vi "4Pi Focus Lock.vi"() -> ()   [LabVIEW 2016]
uses:
  4Pi Focus Lock Controls/4Pi Focus Lock - Notifier Type.ctl
  4Pi Focus Lock Controls/4Pi Focus Lock - Actions.ctl
  <vilib>/vision/Image Controls.llb/IMAQ Image.ctl
  Hardware Configuration/Hardware Configuration Controls/Device Type.ctl
  Hardware Configuration/Hardware Configuration Controls/Device Function.ctl
  Device Library/Cameras/Camera Controls/Generic Camera ROI.ctl
  Device Library/Cameras/Camera Controls/Generic Camera Actions.ctl
  Device Library/Stages/Stages Controls/Stage Actions.ctl
  <vilib>/addons/control/pid/pid.llb/PID (DBL).vi
  <vilib>/addons/control/pid/NI_PID_pid.lvlib
  <vilib>/vision/NI_Vision_Development_Module.lvlib
panel:
  out "CC Max":cluster{" cc max":dbl}(graph)
  in  "Pixe Size (µm)":dbl=2.0
  out "X Y Fit Value (µm)":cluster{dbl, dbl, dbl}(graph)
  out "cc max":dbl=1.0 format="%.3g"
  out "Target X Position cc (px)":dbl=1.0 format="%.3g"
  out "Target Y Position cc (px)":dbl=1.0 format="%.3g"
  out "Measured Y Position cc (px)":dbl=1.0 format="%.3g"
  out "Measured X Position cc (px)":dbl=1.0 format="%.3g"
  in  "Z Correction Active":bool=TRUE
  in  "Frame Accumulation":u32=1
  in  "Z Drift Threshold (µm)":dbl=2.0
  in  "Z Move Limit (µm)":dbl=2.0
  out "Z Move":bool
  in  "Update Scale Factor":dbl=2.0
  out "dz (µm)":dbl format="%.2f"
  out "dt (s)":dbl format="%.3f"
  out "Measured Z (µm)":dbl=1.0 format="%.3g"
  out "Target Z (µm)":dbl=1.0 format="%.3g"
  out "Stage Position (µm)":dbl=1.0 format="%.2g"
  in  "Quit":bool
  in  "Sample Z Step No.":u32=2
  in  "Sample Z Step Size (µm)":dbl=2.0
  in  "D (Derivative)":dbl
  in  "I (Integral)":dbl
  in  "P (Proportional)":dbl=2.0
  in  "Set Camera ROI":bool
  out "Z Target and Fit Value (µm)":T1(graph)
  in  "Start Lock":bool
  # "PID Control Values"
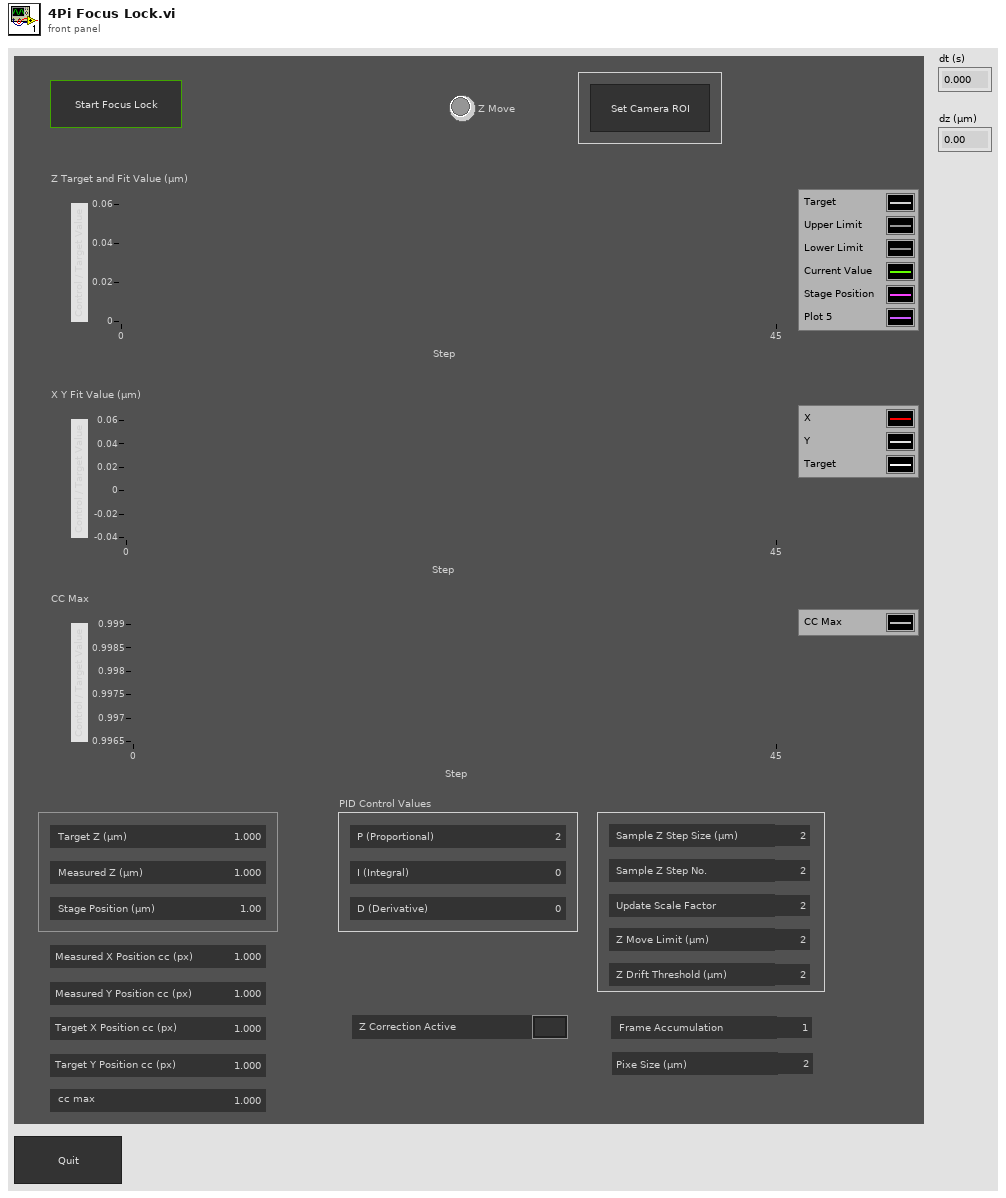
[diagram p1: front panel]
types:
  T1 = cluster{"Target 01":dbl, dbl, dbl, "Current 01":dbl, "Stage Position":dbl}
  T2 = typedef "4Pi Focus Lock - Actions.ctl" = enum16{"Idle", "Start Lock", "Restart Lock", "Get Target Position", "Get Ref Stack", "Cal Ref FFT", "Move To Init Z", "Start Primary Camera", "Get Current Position", "Get Current XY Position", "Get Current Position 1", "Get Actual Position", "Check Drift", "Move Z", "Update Plots", "Delay", "Abort", "Exit Loop", "Quit"}
  T3 = typedef "4Pi Focus Lock - Notifier Type.ctl" = cluster{"Actions":T2, "Z Drift Threshold":dbl, "Z Stage Move Limit (µm)":dbl, "Abort If Error":bool, "Z Correction Active":bool, "PID Values":dbl[], "Running?":bool, "Update Delay (ms)":i32, "Z Step Size (µm)":dbl, "Z Step No.":u32, "No. of Frames":u32, "Ref Stack (SGL)":T4[], "Cur Image (SGL)":T4, "CC Image (SGL) ":T4, "Sample Z (µm)":dbl[], "Initial Z Position (µm)":dbl, "Ref FFT Stack (CSG)":T4[], "Tmp Image FFT (CSG) ":T4[], "CC Image Max (SGL)":T4}
  T4 = typedef "IMAQ Image.ctl" = refnum<image>
  T5 = typedef "Image Type" = u32
  T6 = typedef "Device Function.ctl" = enum16{"Primary", "Secondary", "Overview", "Wide Field Drift Correction", "642 nm Excitation", "560 nm Excitation", "940 nm Excitation", "546 nm Excitation", "488 nm Excitation", "405 nm Excitation", "Objective Drift Correction", "4Pi Focus Lock", "4Pi Objective Lock", "Objective XY", "Objective Z", "Sample XY", "Sample Coarse Z", "Sample Z", "4Pi Lower", "4Pi Upper", "Em Small", "Em Large", "Ex Small", "Ex Large", "Mojo", "Adj Cavity", "Line Scanning", "Alert"}
  T7 = typedef "Device Type.ctl" = enum16{"AOTF", "Camera", "Deformable Mirror", "Laser", "Flip Mirror", "Shutter", "Stage", "Waveform", "FPGA", "Email"}
  T8 = typedef "Stage Actions.ctl" = enum16{"Get Position", "MVR", "MOVE", "HALT", "ONTARGET", "ERROR", "REFERENCE", "INIT", "VELOCITY", "STATUS", "EXIT", "HOME", "ZEROPOS", "NANOPOS", "ANALOG", "QUIT"}
  T9 = typedef "Generic Camera Actions.ctl" = enum16{"Status", "Live Preview", "Capture", "Abort", "Set Exposure Time (s)", "Get Exposure Time (s)", "Record Settings", "Set ROI", "Get ROI", "Defect Correction On/Off", "Cooler On/Off", "Fan On/Off", "Quit"}
  T10 = typedef "Generic Camera ROI.ctl" = cluster{"H_Offset":u16, "V_Offset":u16, "H_Width":u16, "V_Width":u16}
  T11 = typedef "Stage Status.ctl" = enum16{"Error", "Abort", "Busy", "On Target"}
  T12 = typedef "2D Gaussian - Best Fit Parameters.ctl" = cluster{"Amplitude":dbl, "X Position":dbl, "Y Position":dbl, "X Width":dbl, "Y Width":dbl, "Offset":dbl}
  T13 = cluster{"PID Values[0]":dbl, "PID Values[1]":dbl, "PID Values[2]":dbl}
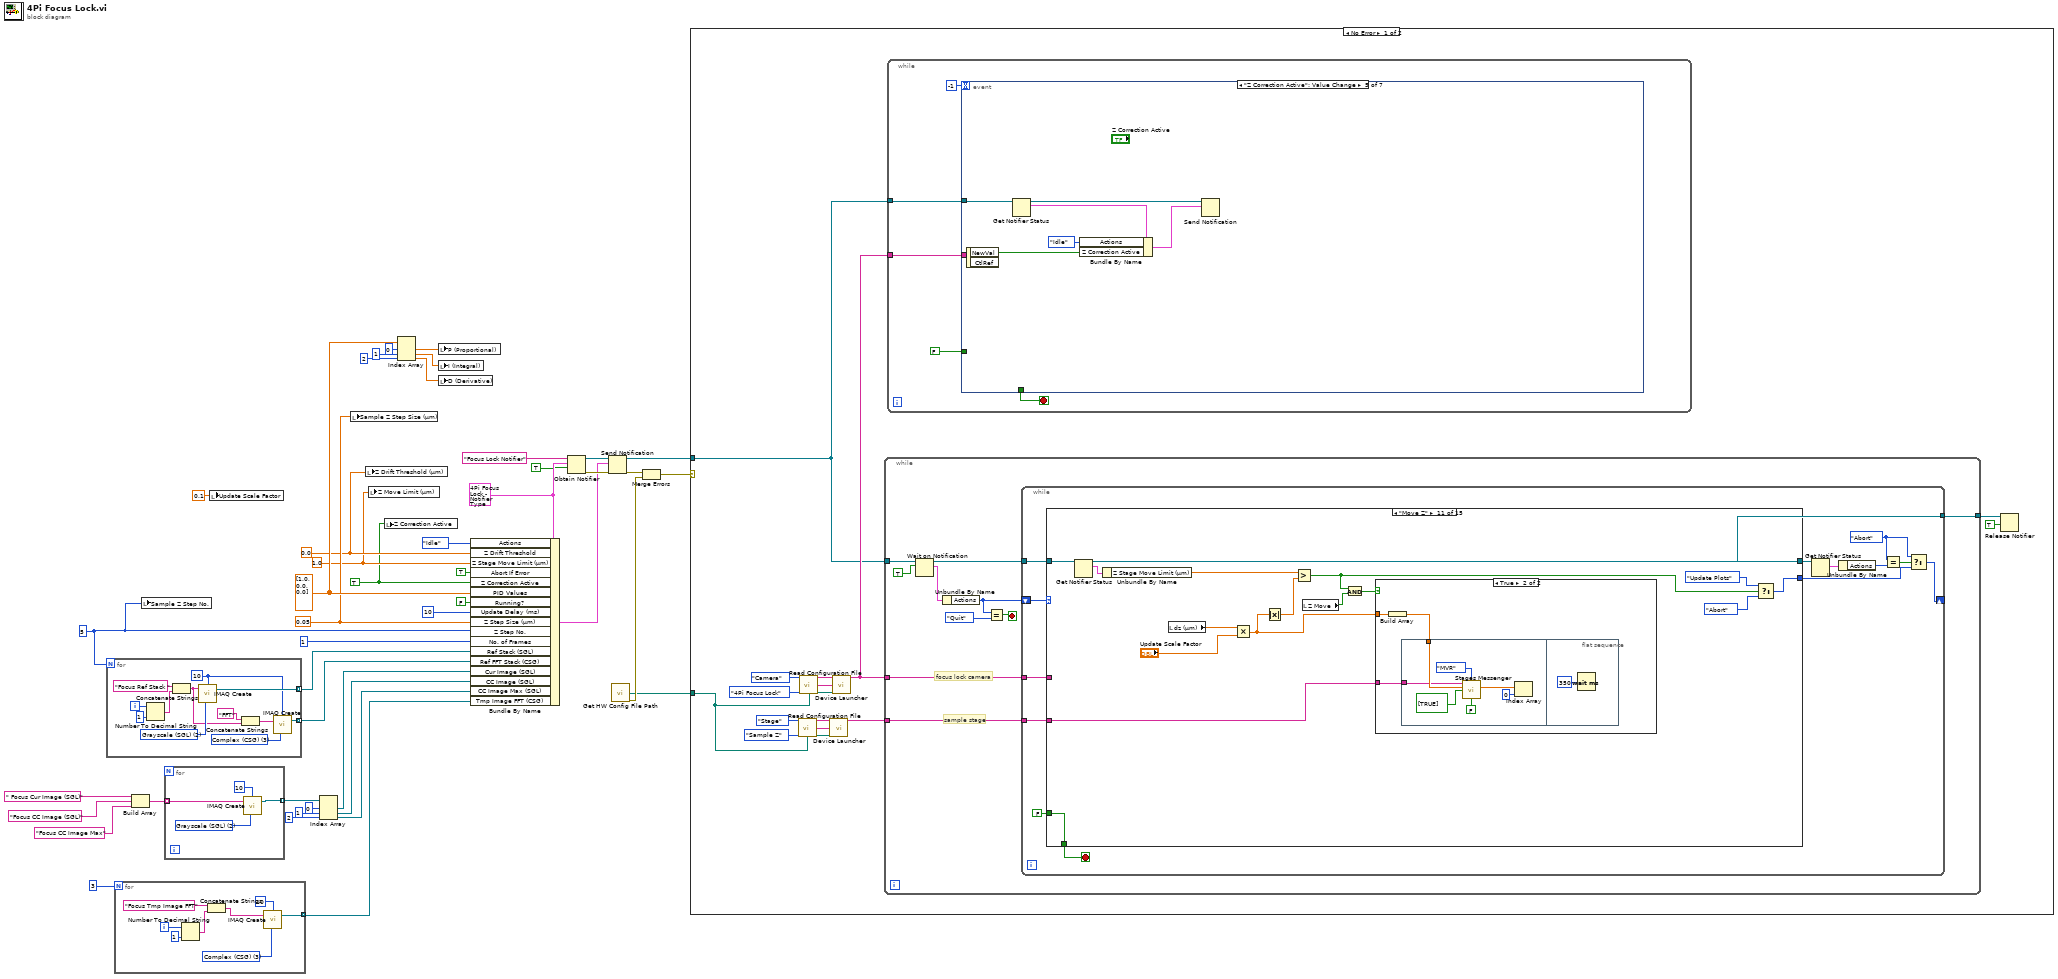
[diagram p0: block diagram]
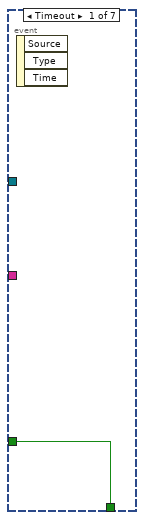
[diagram p2: hidden frame]
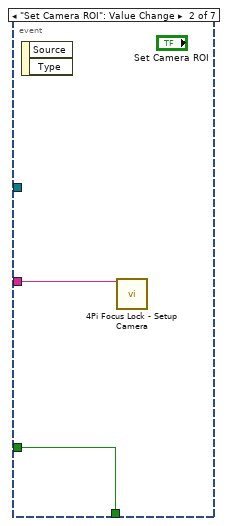
[diagram p3: hidden frame]
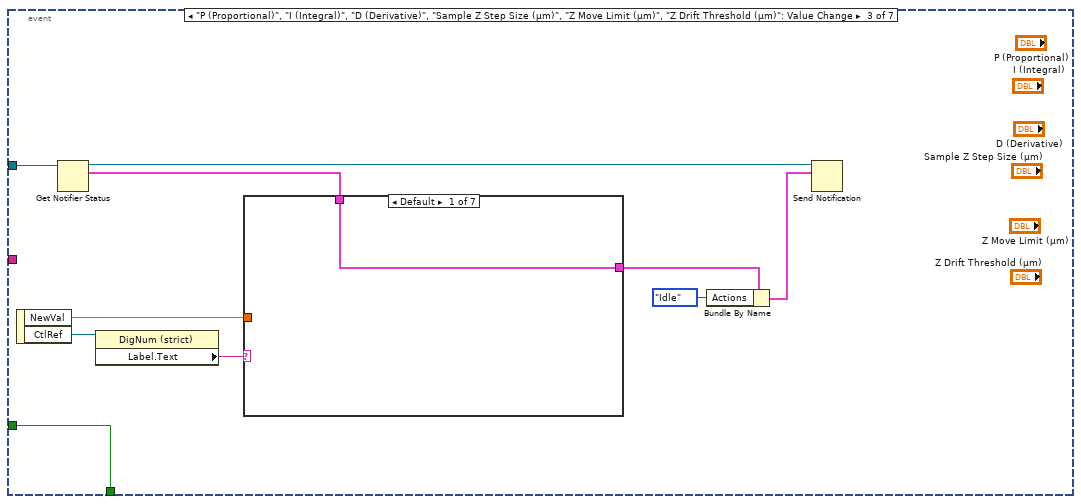
[diagram p4: hidden frame]
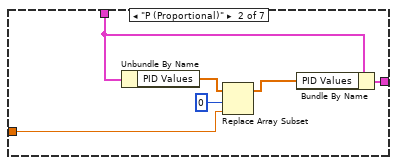
[diagram p5: hidden frame]
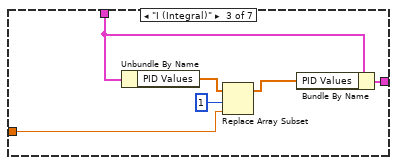
[diagram p6: hidden frame]
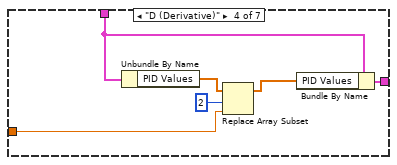
[diagram p7: hidden frame]
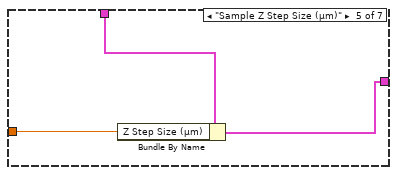
[diagram p8: hidden frame]
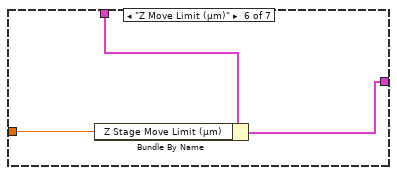
[diagram p9: hidden frame]
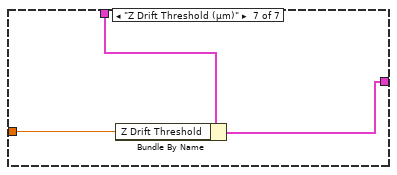
[diagram p10: hidden frame]
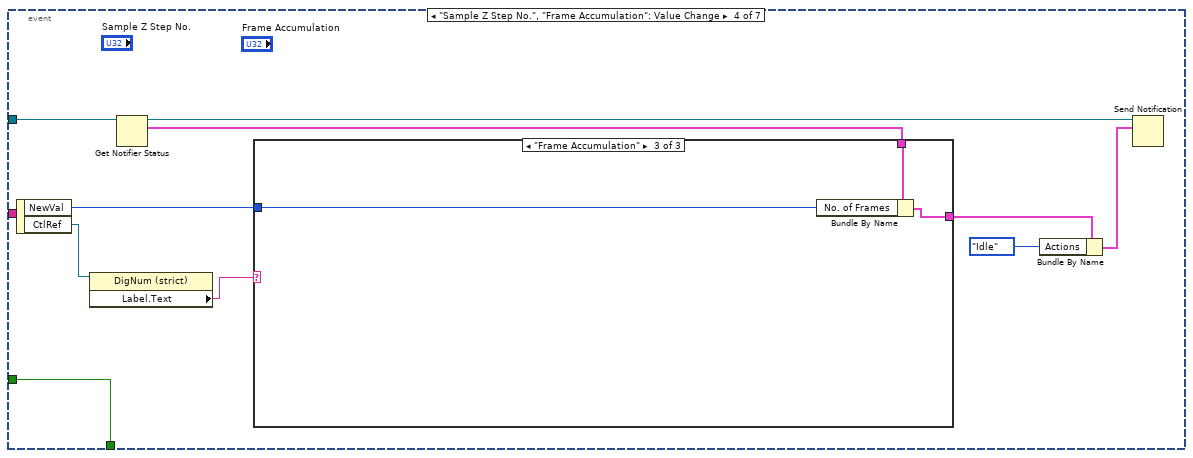
[diagram p11: hidden frame]
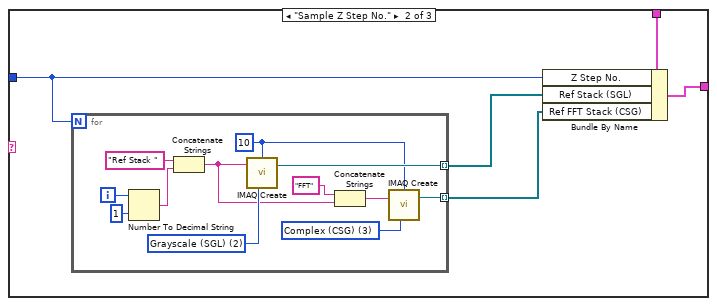
[diagram p13: hidden frame]
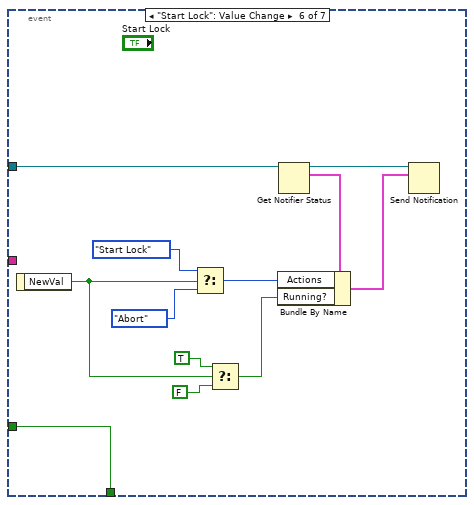
[diagram p14: hidden frame]
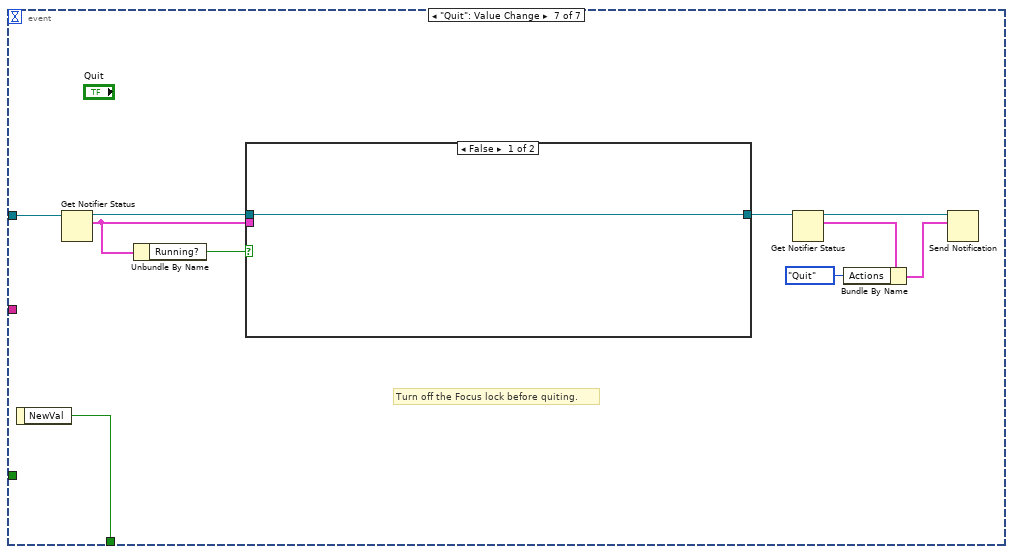
[diagram p15: hidden frame]
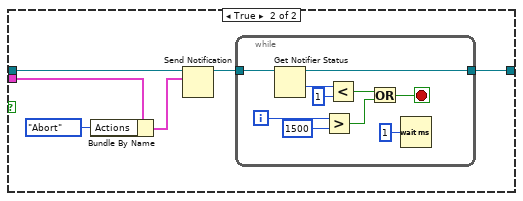
[diagram p16: hidden frame]
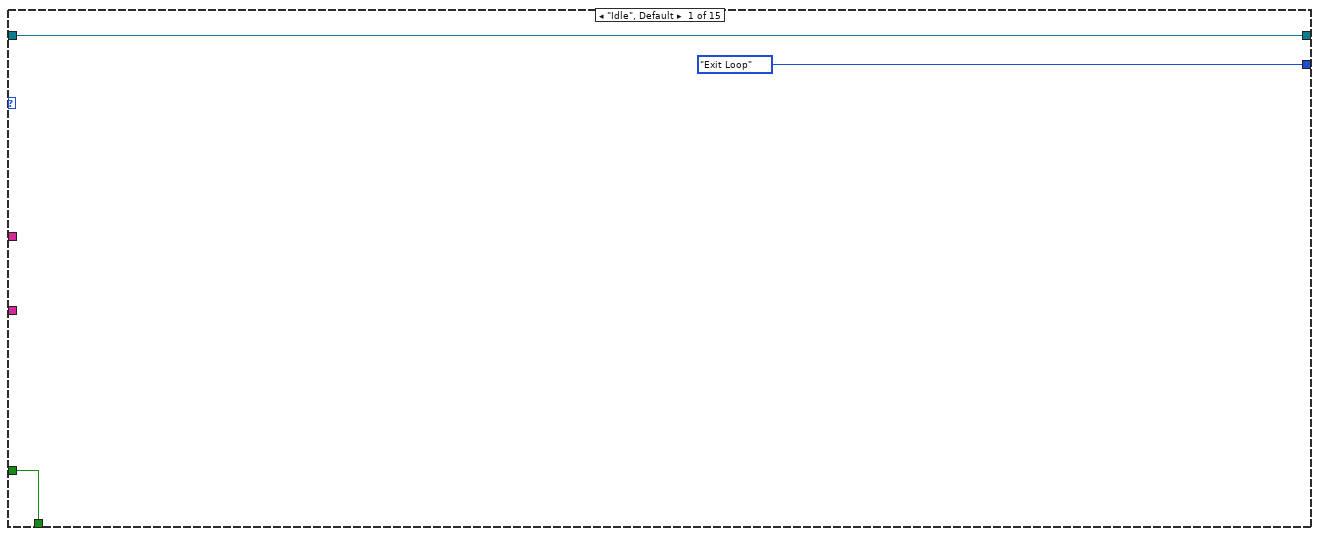
[diagram p17: hidden frame]
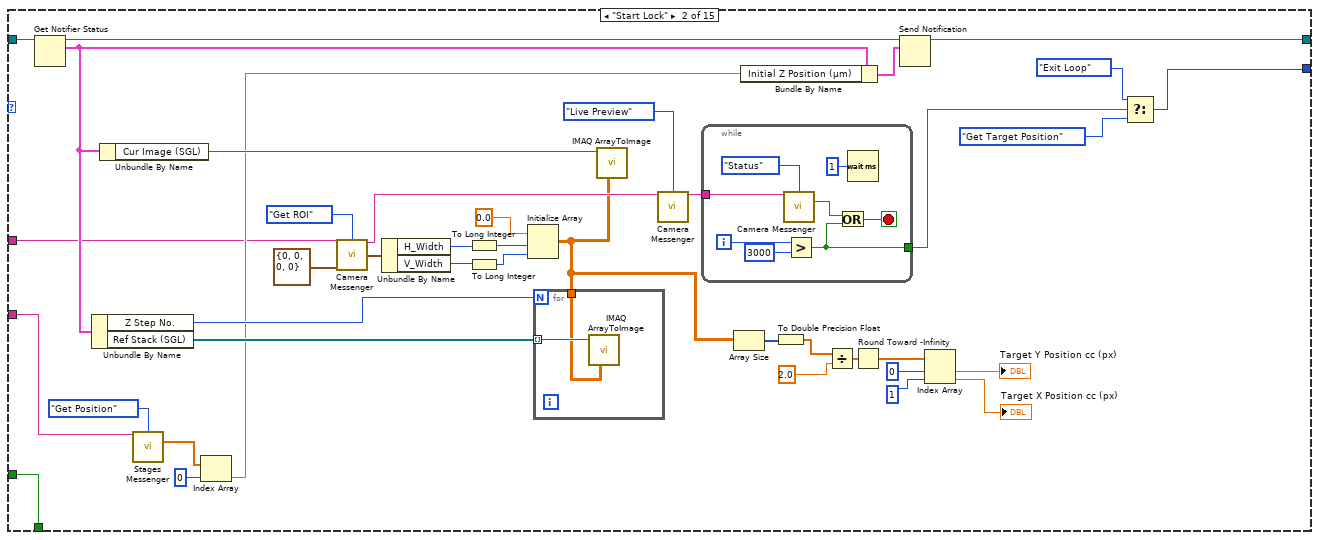
[diagram p18: hidden frame]
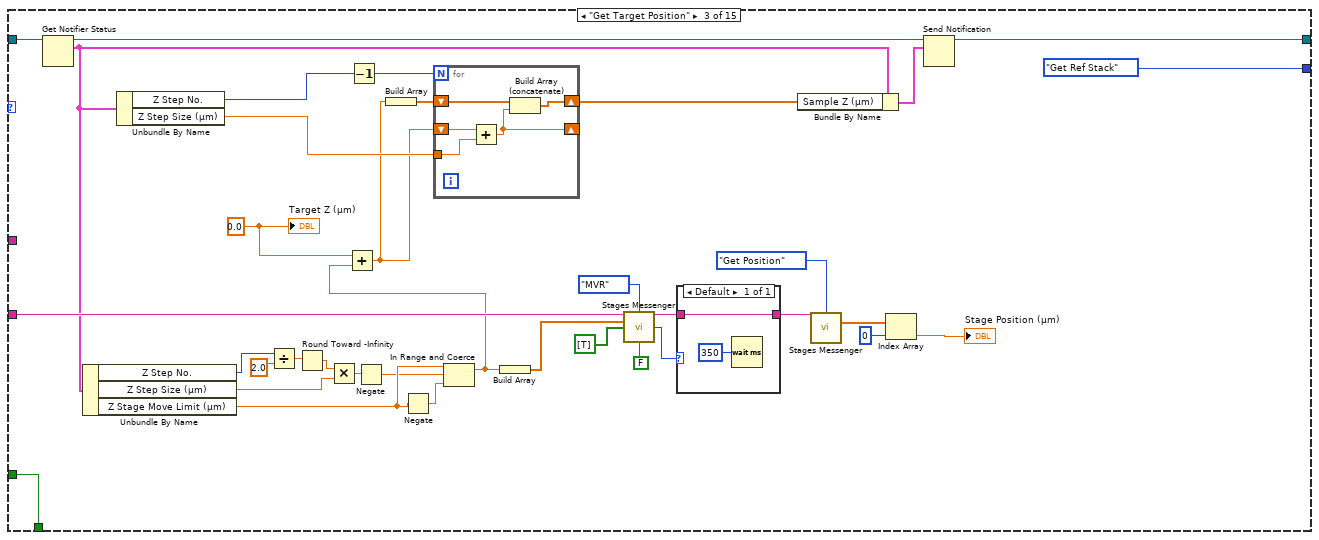
[diagram p19: hidden frame]
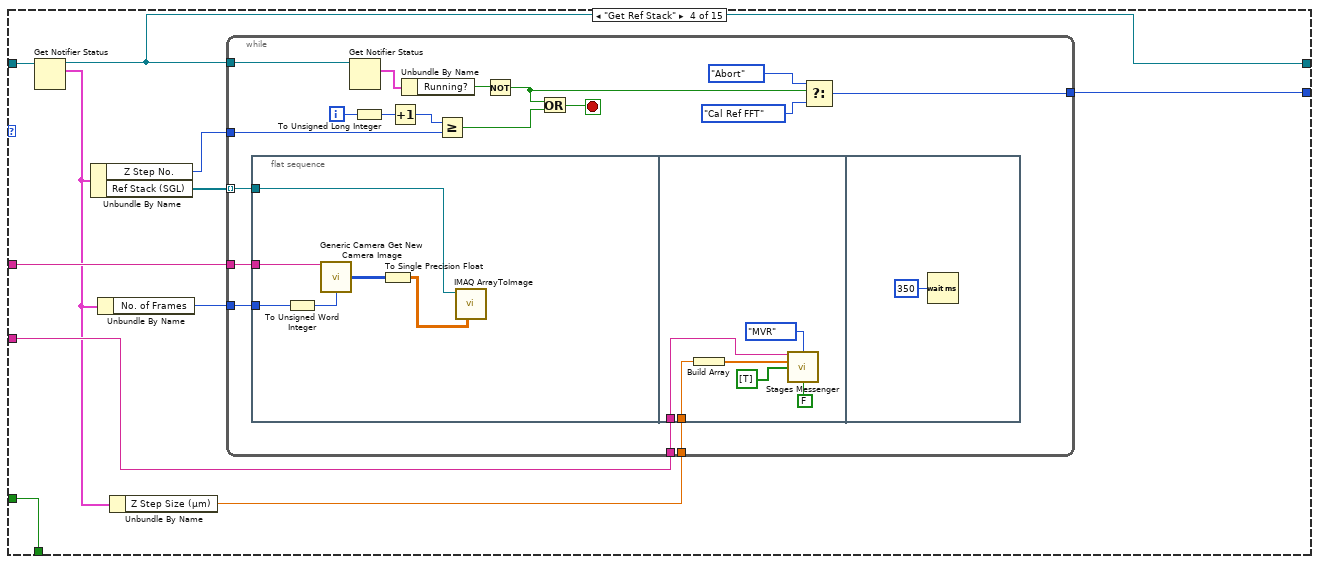
[diagram p20: hidden frame]
diagram:
  w23 = u32 5 ("Z Step No.")
  w30 = 0.05 ("Z Step Size (µm)")
  w34 = dbl[] [1.0, 0.0, 0.0] ("PID Values")
  w4 = TRUE ("Z Correction Active")
  w10 = 1.0 ("Z Stage Move Limit (µm)")
  w11 = 0.0 ("Z Drift Threshold")
  w13 = T3 {"Actions"=enum."Idle", "Z Drift Threshold"=0.05, "Z Stage Move Limit (µm)"=1.0, "Abort If Error"=FALSE, "Z Correction Active"=FALSE, "PID Values"=[], "Running?"=FALSE, "Update Delay (ms)"=0, "Z Step Size (µm)"=2.0, "Z Step No."=2, "No. of Frames"=0, "Ref Stack (SGL)"=[], "Cur Image (SGL)"=refnum, "CC Image (SGL) "=refnum, "Sample Z (µm)"=[], "Initial Z Position (µm)"=0.0, "Ref FFT Stack (CSG)"=[], "Tmp Image FFT (CSG) "=[], "CC Image Max (SGL)"=refnum} ("4Pi Focus Lock")
  n1 = for {
    N: w23 -> [_]
    tunnel: [w56] -> w22 mode=indexing
    tunnel: [w45] -> w7 mode=indexing
    i -> [w55]
    w50 = T5 3 items=["Grayscale (U8)", "Grayscale (I16)", "Grayscale (SGL)", "Complex (CSG)", "RGB (U32)", "HSL (U32)", "RGB (U64)", "Grayscale (U16)"] ("Image Type")
    w51 = T5 2 items=["Grayscale (U8)", "Grayscale (I16)", "Grayscale (SGL)", "Complex (CSG)", "RGB (U32)", "HSL (U32)", "RGB (U64)", "Grayscale (U16)"] ("Image Type")
    w47 = 10 ("Border Size")
    n2 = Number To Decimal String(number=w55, width (-)=i16 1) -> (decimal integer string=w53:string)
    n3 = Concatenate Strings("Focus Ref Stack " ("string"), w53) -> (w46:string)
    n4 = call "IMAQ Create"("Border Size"=w47, "Image Name"=w46, "Image Type"=w51) -> ("New Image"=w56:T4)  [unwired: 2 in, 1 out]
    n5 = Concatenate Strings("FFT" ("string"), w46) -> (w49:string)
    n6 = call "IMAQ Create"("Border Size"=w47, "Image Name"=w49, "Image Type"=w50) -> ("New Image"=w45:T4)  [unwired: 2 in, 1 out]
  }
  n7 = for {
    N: 3 -> [_]
    tunnel: [w62] -> w5 mode=indexing
    i -> [w58]
    w63 = T5 3 items=["Grayscale (U8)", "Grayscale (I16)", "Grayscale (SGL)", "Complex (CSG)", "RGB (U32)", "HSL (U32)", "RGB (U64)", "Grayscale (U16)"] ("Image Type")
    n8 = Number To Decimal String(number=w58, width (-)=i16 1) -> (decimal integer string=w61:string)
    n9 = Concatenate Strings("Focus Tmp Image FFT" ("Image Name"), w61) -> (w57:string)
    n10 = call "IMAQ Create"("Border Size"=10, "Image Name"=w57, "Image Type"=w63) -> ("New Image"=w62:T4)  [unwired: 2 in, 1 out]
  }
  n11 = Build Array(" Focus Cur Image (SGL)" ("Image Name"), "Focus CC Image (SGL)" ("Image Name"), "Focus CC Image Max" ("element")) -> (w17:string[])
  n12 = local write "Sample Z Step No."(w23) -> ()
  n13 = for {
    tunnel: w17 -> [w66] mode=indexing
    tunnel: [w65] -> w16 mode=indexing
    w67 = T5 2 items=["Grayscale (U8)", "Grayscale (I16)", "Grayscale (SGL)", "Complex (CSG)", "RGB (U32)", "HSL (U32)", "RGB (U64)", "Grayscale (U16)"] ("Image Type")
    n14 = call "IMAQ Create"("Border Size"=10, "Image Name"=w66, "Image Type"=w67) -> ("New Image"=w65:T4)  [unwired: 2 in, 1 out]
  }
  n15 = local write "Update Scale Factor"(0.1 ("Update Scale Factor")) -> ()
  n16 = Index Array(array=w16, index #1=0 ("index"), index #2=1 ("index"), index #3=2 ("index")) -> (element #1=w15:T4, element #2=w14:T4, element #3=w1:T4)
  n17 = local write "Sample Z Step Size (µm)"(w30) -> ()
  n18 = local write "Z Drift Threshold (µm)"(w11) -> ()
  n19 = local write "Z Move Limit (µm)"(w10) -> ()
  n20 = local write "Z Correction Active"(w4) -> ()
  n21 = Index Array(array=w34, index #1=0 ("index"), index #2=1 ("index"), index #3=2 ("index")) -> (element #1=w33:dbl, element #2=w32:dbl, element #3=w31:dbl)
  n22 = local write "P (Proportional)"(w33) -> ()
  n23 = local write "I (Integral)"(w32) -> ()
  n24 = local write "D (Derivative)"(w31) -> ()
  n25 = Bundle By Name(cluster=w13, "Actions"=4Pi_Focus_Lock_-_Actions."Idle", "Z Drift Threshold"=w11, "Z Stage Move Limit (µm)"=w10, "Abort If Error"=TRUE, "Z Correction Active"=w4, "PID Values"=w34, "Running?"=FALSE, "Update Delay (ms)"=10, "Z Step Size (µm)"=w30, "Z Step No."=w23, "No. of Frames"=u32 1, "Ref Stack (SGL)"=w22, "Ref FFT Stack (CSG)"=w7, "Cur Image (SGL)"=w15, "CC Image (SGL)"=w14, "CC Image Max (SGL)"=w1, "Tmp Image FFT (CSG)"=w5) -> (w8:T3)
  n26 = Obtain Notifier(name (unnamed)="Focus Lock Notifier", notification data type=w13, create if not found? (T)=TRUE) -> (notifier out=w39:refnum<notifier>, error out=w38:errorcluster)  [unwired: 1 in, 1 out]
  n27 = Send Notification(notification=w8, notifier=w39, error in (no error)=w38) -> (notifier out=w25:refnum<notifier>, error out=w29:errorcluster)
  n28 = call "Get HW Config File Path.vi"() -> ("File Path"=w27:path, "Error"=w28:errorcluster)  [unwired: 14 in]
  n29 = Merge Errors(w29, w28) -> (w26:errorcluster)
  n30 = case shown="No Error" w26 {
    tunnel: w27 -> [w69 _]
    tunnel: w25 -> [w72 _]
    frame No Error {
      n31 = call "Read Configuration File.vi"("Device Type"=Device_Type."Stage", "Device Function"=Device_Function."Sample Z", "Config File Path"=w69) -> ("Unique Notifier Name"=w79:string, "Device Ports/IDs/Channels"=w77:string[], "Device Engine Path"=w76:path)  [unwired: 9 in, 1 out]
      n32 = call "Read Configuration File.vi"("Device Type"=Device_Type."Camera", "Device Function"=Device_Function."4Pi Focus Lock", "Config File Path"=w69) -> ("Unique Notifier Name"=w84:string, "Device Ports/IDs/Channels"=w83:string[], "Device Engine Path"=w82:path)  [unwired: 9 in, 1 out]
      n33 = call "Device Launcher.vi"("Notifier Name"=w79, "Device Ports/IDs/Channels"=w77, "Device Engine Path"=w76) -> ("Notifier Name"=w74:string)  [unwired: 11 in, 1 out]
      n34 = call "Device Launcher.vi"("Notifier Name"=w84, "Device Ports/IDs/Channels"=w83, "Device Engine Path"=w82) -> ("Notifier Name"=w73:string)  [unwired: 11 in, 1 out]
      n35 = while {
        tunnel: w72 -> [w216]
        tunnel: w73 -> [w210]
        tunnel: w74 -> [w209]
        tunnel: [w207] -> w70
        stop <- w212 stop-if-true
        # "sample stage"
        # "focus lock camera"
        n36 = Wait on Notification(notifier=w216, ignore previous (F)=TRUE) -> (notifier out=w208:refnum<notifier>, notification=w214:T3)  [unwired: 2 in, 2 out]
        n37 = Unbundle By Name(w214) -> ("Actions"=w211:T2)
        n38 = Equal?(x=w211, y=4Pi_Focus_Lock_-_Actions."Quit") -> (x = y?=w212:bool)
        n39 = while {
          tunnel: w210 -> [w228]
          tunnel: w209 -> [w227]
          tunnel: w208 -> [w226]
          shift-right: [w220] -> _
          shift-left: w211 -> [w229]
          tunnel: [w217] -> w207
          stop <- w219 stop-if-true
          w222 = 4Pi_Focus_Lock_-_Actions."Abort" ("y")
          n40 = case shown="\"Move Z\"" w229 {
            tunnel: w228 -> [_ w249 _ w335 _ _ w421 _ w478 _ _ _ w592 _ _]
            tunnel: w227 -> [_ w256 w313 w328 _ w380 _ _ _ _ w537 w575 _ _ _]
            tunnel: w226 -> [w230 w265 w314 w336 w373 w385 w434 w453 w493 w522 w542 w585 w593 w600 w603]
            tunnel: [4Pi_Focus_Lock_-_Actions."Exit Loop" ("y") w243 4Pi_Focus_Lock_-_Actions."Get Ref Stack" ("y") w329 4Pi_Focus_Lock_-_Actions."Move To Init Z" ("y") 4Pi_Focus_Lock_-_Actions."Get Current Position" ("y") w424 4Pi_Focus_Lock_-_Actions."Check Drift" ("y") 4Pi_Focus_Lock_-_Actions."Check Drift" ("y") w505 w527 4Pi_Focus_Lock_-_Actions."Get Current Position" ("y") 4Pi_Focus_Lock_-_Actions."Exit Loop" ("y") 4Pi_Focus_Lock_-_Actions."Exit Loop" ("y") 4Pi_Focus_Lock_-_Actions."Quit" ("y")] -> w221
            tunnel: [w230 w251 w301 w331 w370 w383 w431 w449 w488 w515 w535 w573 w589 w600 w603] -> w217
            tunnel: [w231 w250 w300 w330 w368 w381 w430 w447 w487 w514 w534 w572 w588 TRUE TRUE] -> w219
            tunnel: FALSE -> [w231 w250 w300 w330 w368 w381 w430 w447 w487 w514 w534 w572 w588 _ _]
            frame "Idle", Default {
            }
            frame "Start Lock" {
              n41 = Get Notifier Status(notifier=w265) -> (notifier out=w252:refnum<notifier>, current notification=w255:T3)  [unwired: 1 in, 3 out]
              n42 = Unbundle By Name(w255) -> ("Z Step No."=w262:u32, "Ref Stack (SGL)"=w261:T4[])
              n43 = Unbundle By Name(w255) -> ("Cur Image (SGL)"=w260:T4)
              n44 = call "Stages Messenger.vi"("Stage Notifier Name"=w256, "Actions"=Stage_Actions."Get Position") -> ("Positions"=w257:dbl[])  [unwired: 10 in, 3 out]
              n45 = Index Array(array=w257, index=0) -> (element=w254:dbl)
              n46 = call "Camera Messenger.vi"("Notifier Name"=w249, "General Camera Actions"=Generic_Camera_Actions."Get ROI", "Camera ROI"=T10 {"H_Offset"=0, "V_Offset"=0, "H_Width"=0, "V_Width"=0} ("General Camera ROI")) -> ("Notifier Name Dup"=w248:string, "Camera ROI"=w270:T10)  [unwired: 7 in, 4 out]
              n47 = Unbundle By Name(w270) -> ("H_Width"=w269:u16, "V_Width"=w267:u16)
              n48 = To Long Integer(number=w269) -> (32bit integer=w268:i32)
              n49 = To Long Integer(number=w267) -> (32bit integer=w266:i32)
              n50 = Initialize Array(sgl 0.0 ("element"), w268, w266) -> (w233:sgl[][])
              n51 = for {
                N: w262 -> [_]
                tunnel: w233 -> [w281]
                tunnel: w261 -> [w282] mode=indexing
                n52 = call "IMAQ ArrayToImage"("Image Pixels (Float)"=w281, "Image"=w282) -> ()  [unwired: 8 in, 2 out]
              }
              n53 = call "IMAQ ArrayToImage"("Image Pixels (Float)"=w233, "Image"=w260) -> ()  [unwired: 8 in, 2 out]
              n54 = call "Camera Messenger.vi"("Notifier Name"=w248, "General Camera Actions"=Generic_Camera_Actions."Live Preview") -> ("Notifier Name Dup"=w247:string)  [unwired: 8 in, 5 out]
              n55 = while {
                tunnel: w247 -> [w279]
                tunnel: [w274] -> w246
                i -> [w278]
                stop <- w275 stop-if-true
                n56 = call "Camera Messenger.vi"("Notifier Name"=w279, "General Camera Actions"=Generic_Camera_Actions."Status") -> ("Running?"=w276:bool)  [unwired: 8 in, 5 out]
                n57 = Greater?(x=w278, y=3000) -> (0:w274:bool)
                n58 = Or(x=w276, y=w274) -> (x .or. y?=w275:bool)
                n59 = Wait (ms)(milliseconds to wait=u32 1) -> ()  [unwired: 1 out]
              }
              n60 = Array Size(array=w233) -> (size(s)=w239:i32[])
              n61 = Bundle By Name(cluster=w255, "Initial Z Position (µm)"=w254) -> (w253:T3)
              n62 = To Double Precision Float(number=w239) -> (double precision float=w242:dbl[])
              n63 = Divide(x=w242, y=2.0 ("index")) -> (x/y=w240:dbl[])
              n64 = Round Toward -Infinity(1:w240) -> (0:w238:dbl[])
              n65 = Send Notification(notification=w253, notifier=w252) -> (notifier out=w251:refnum<notifier>)  [unwired: 1 in, 1 out]
              n66 = Index Array(array=w238, index #1=0 ("index"), index #2=1 ("index")) -> (element #1=→"Target Y Position cc (px)":dbl, element #2=→"Target X Position cc (px)":dbl)
              n67 = Select(t=4Pi_Focus_Lock_-_Actions."Exit Loop" ("y"), s=w246, f=4Pi_Focus_Lock_-_Actions."Get Target Position") -> (s? t:f=w243:T2)
            }
            frame "Get Target Position" {
              w307 = 0.0 ("Target Z (µm)")
              n68 = Get Notifier Status(notifier=w314) -> (notifier out=w305:refnum<notifier>, current notification=w310:T3)  [unwired: 1 in, 3 out]
              n69 = Unbundle By Name(w310) -> ("Z Step No."=w299:u32, "Z Step Size (µm)"=w298:dbl, "Z Stage Move Limit (µm)"=w296:dbl)
              n70 = Unbundle By Name(w310) -> ("Z Step No."=w291:u32, "Z Step Size (µm)"=w308:dbl)
              n71 = Divide(x=w299, y=2.0) -> (x/y=w289:dbl)
              n72 = Round Toward -Infinity(1:w289) -> (0:w288:dbl)
              n73 = Multiply(x=w288, y=w298) -> (x*y=w293:dbl)
              n74 = Decrement(x=w291) -> (x-1=w290:u32)
              n75 = Negate(x=w293) -> (-x=w292:dbl)
              n76 = Negate(x=w296) -> (-x=w297:dbl)
              n77 = In Range and Coerce(upper limit=w296, x=w292, lower limit=w297) -> (coerced(x)=w294:dbl)  [unwired: 1 out]
              n78 = Add(x=w307, y=w294) -> (x+y=w295:dbl)
              n79 = Build Array(w295) -> (w309:dbl[])
              n80 = for {
                N: w290 -> [_]
                tunnel: w308 -> [w323]
                shift-right: [w324] -> w306
                shift-left: w309 -> [w325]
                shift-right: [w321] -> _
                shift-left: w295 -> [w322]
                n81 = Add(x=w322, y=w323) -> (x+y=w321:dbl)
                n82 = Build Array (concatenate)(w325, w321) -> (w324:dbl[])
              }
              n83 = Build Array(w294) -> (w311:dbl[])
              n84 = call "Stages Messenger.vi"("Stage Notifier Name"=w313, "Actions"=Stage_Actions."MVR", "Setpoint"=w311, "Axis"=bool[] [TRUE], "Exit While Busy?"=FALSE) -> ("Stage Notifier Name (Dup)"=w286:string, "Status"=w287:T11)  [unwired: 7 in, 2 out]
              n85 = case shown="Default" w287 {
                tunnel: [w319] -> w285
                tunnel: w286 -> [w319]
                frame Default {
                  n86 = Wait (ms)(milliseconds to wait=u32 350) -> ()  [unwired: 1 out]
                }
              }
              n87 = Bundle By Name(cluster=w310, "Sample Z (µm)"=w306) -> (w304:T3)
              n88 = call "Stages Messenger.vi"("Stage Notifier Name"=w285, "Actions"=Stage_Actions."Get Position") -> ("Positions"=w283:dbl[])  [unwired: 10 in, 3 out]
              n89 = Index Array(array=w283, index=0) -> (element=→"Stage Position (µm)":dbl)
              n90 = Send Notification(notification=w304, notifier=w305) -> (notifier out=w301:refnum<notifier>)  [unwired: 1 in, 1 out]
              "Target Z (µm)" <- w307
            }
            frame "Get Ref Stack" {
              n91 = Get Notifier Status(notifier=w336) -> (notifier out=w331:refnum<notifier>, current notification=w327:T3)  [unwired: 1 in, 3 out]
              n92 = Unbundle By Name(w327) -> ("Z Step No."=w334:u32, "Ref Stack (SGL)"=w333:T4[])
              n93 = Unbundle By Name(w327) -> ("No. of Frames"=w326:u32)
              n94 = Unbundle By Name(w327) -> ("Z Step Size (µm)"=w332:dbl)
              n95 = while {
                tunnel: w335 -> [w354]
                tunnel: w334 -> [w351]
                tunnel: w331 -> [w353]
                tunnel: [w341] -> w329
                tunnel: w333 -> [w340] mode=indexing
                tunnel: w332 -> [w339]
                tunnel: w328 -> [w338]
                tunnel: w326 -> [w337]
                i -> [w350]
                stop <- w346 stop-if-true
                n96 = flat-sequence {
                  tunnel: w354 -> [w358]
                  tunnel: w340 -> [w357]
                  tunnel: w337 -> [w356]
                  tunnel: w339 -> [w362]
                  tunnel: w338 -> [w361]
                  frame #0 {
                    n97 = To Unsigned Word Integer(number=w356) -> (unsigned 16bit integer=w355:u16)
                    n98 = call "Generic Camera Get New Camera Image.vi"("Camera Notifier Name"=w358, "Frames"=w355) -> ("Image - U16"=w360:u16[][])  [unwired: 11 in, 2 out]
                    n99 = To Single Precision Float(number=w360) -> (single precision float=w359:sgl[][])
                    n100 = call "IMAQ ArrayToImage"("Image Pixels (Float)"=w359, "Image"=w357) -> ()  [unwired: 8 in, 2 out]
                  }
                  frame #1 {
                    n101 = Build Array(w362) -> (w366:dbl[])
                    n102 = call "Stages Messenger.vi"("Stage Notifier Name"=w361, "Actions"=Stage_Actions."MVR", "Setpoint"=w366, "Axis"=bool[] [TRUE], "Exit While Busy?"=FALSE) -> ()  [unwired: 7 in, 4 out]
                  }
                  frame #2 {
                    n103 = Wait (ms)(milliseconds to wait=u32 350) -> ()  [unwired: 1 out]
                  }
                }
                n104 = Get Notifier Status(notifier=w353) -> (current notification=w345:T3)  [unwired: 1 in, 4 out]
                n105 = To Unsigned Long Integer(number=w350) -> (unsigned 32bit integer=w349:u32)
                n106 = Increment(x=w349) -> (x+1=w352:u32)
                n107 = Unbundle By Name(w345) -> ("Running?"=w348:bool)
                n108 = Greater Or Equal?(x=w352, y=w351) -> (x >= y?=w347:bool)
                n109 = Not(x=w348) -> (.not. x?=w344:bool)
                n110 = Or(x=w344, y=w347) -> (x .or. y?=w346:bool)
                n111 = Select(t=4Pi_Focus_Lock_-_Actions."Abort", s=w344, f=4Pi_Focus_Lock_-_Actions."Cal Ref FFT" ("y")) -> (s? t:f=w341:T2)
              }
            }
            frame "Cal Ref FFT" {
              n112 = Get Notifier Status(notifier=w373) -> (notifier out=w370:refnum<notifier>, current notification=w374:T3)  [unwired: 1 in, 3 out]
              n113 = Unbundle By Name(w374) -> ("Ref Stack (SGL)"=w371:T4[], "Ref FFT Stack (CSG)"=w372:T4[])
              n114 = for {
                tunnel: w372 -> [w375] mode=indexing
                tunnel: w371 -> [w376] mode=indexing
                n115 = call "4Pi Focus Lock - Norm FFT.vi"("FFT Image Dst"=w375, "Image In"=w376) -> ()  [unwired: 8 in, 2 out]
              }
            }
            frame "Move To Init Z" {
              n116 = Get Notifier Status(notifier=w385) -> (notifier out=w383:refnum<notifier>, current notification=w384:T3)  [unwired: 1 in, 3 out]
              n117 = Unbundle By Name(w384) -> ("Initial Z Position (µm)"=w378:dbl)
              n118 = flat-sequence {
                tunnel: w380 -> [w393]
                tunnel: [w392] -> w379
                tunnel: w378 -> [w388]
                tunnel: [w386] -> w377
                tunnel: w379 -> [w396]
                tunnel: w377 -> [w395]
                frame #0 {
                  n119 = call "Stages Messenger.vi"("Stage Notifier Name"=w393, "Actions"=Stage_Actions."Get Position") -> ("Stage Notifier Name (Dup)"=w392:string, "Positions"=w390:dbl[])  [unwired: 10 in, 2 out]
                  n120 = Index Array(array=w390, index=0) -> (element=w389:dbl)
                  n121 = Subtract(x=w388, y=w389) -> (x-y=w387:dbl)
                  n122 = Build Array(w387) -> (w386:dbl[])
                }
                frame #1 {
                  n123 = call "Stages Messenger.vi"("Stage Notifier Name"=w396, "Actions"=Stage_Actions."MVR", "Setpoint"=w395, "Axis"=bool[] [TRUE], "Exit While Busy?"=FALSE) -> ()  [unwired: 7 in, 4 out]
                }
                frame #2 {
                  n124 = Wait (ms)(milliseconds to wait=u32 350) -> ()  [unwired: 1 out]
                }
              }
            }
            frame "Get Current Position" {
              n125 = Get Notifier Status(notifier=w434) -> (notifier out=w431:refnum<notifier>, current notification=w418:T3)  [unwired: 1 in, 3 out]
              n126 = Unbundle By Name(w418) -> ("CC Image (SGL)"=w406:T4, "CC Image Max (SGL)"=w401:T4)
              n127 = Unbundle By Name(w418) -> ("Ref FFT Stack (CSG)"=w409:T4[])
              n128 = Unbundle By Name(w418) -> ("No. of Frames"=w412:u32, "Cur Image (SGL)"=w420:T4, "Tmp Image FFT (CSG)"=w414:T4[])
              n129 = Unbundle By Name(w418) -> ("Sample Z (µm)"=w433:dbl[])
              n130 = To Unsigned Word Integer(number=w412) -> (unsigned 16bit integer=w411:u16)
              n131 = call "Generic Camera Get New Camera Image.vi"("Camera Notifier Name"=w421, "Frames"=w411) -> ("Image - U16"=w423:u16[][])  [unwired: 11 in, 2 out]
              n132 = Index Array(array=w414, index #1=0 ("index"), index #2=1 ("index"), index #3=2 ("index")) -> (element #1=w413:T4, element #2=w410:T4, element #3=w407:T4)
              n133 = To Single Precision Float(number=w423) -> (single precision float=w422:sgl[][])
              n134 = call "IMAQ ArrayToImage"("Image Pixels (Float)"=w422, "Image"=w420) -> ("Image Out"=w419:T4)  [unwired: 8 in, 1 out]
              n135 = call "4Pi Focus Lock - Norm FFT.vi"("FFT Image Dst"=w413, "Image In"=w419) -> ("FFT Image Out"=w429:T4)  [unwired: 8 in, 1 out]
              n136 = call "IMAQ ComplexConjugate"("Image Src"=w429) -> ("Image Dst Out"=w408:T4)  [unwired: 3 in, 1 out]
              n137 = for {
                tunnel: [w442] -> w404 mode=indexing
                shift-right: [w442] -> _
                shift-left: sgl 0.0 ("Max CC") -> [w443]
                tunnel: w406 -> [w436]
                tunnel: w410 -> [w440]
                tunnel: w409 -> [w439] mode=indexing
                tunnel: w408 -> [w438]
                tunnel: w407 -> [w437]
                tunnel: w401 -> [w435]
                n138 = call "4Pi Focus Lock - Get Cross Correlation.vi"("Ref FFT image"=w439, "Cur FFT Image"=w438, "FFT CC image"=w440, "iFFT image"=w437, "CC image"=w436) -> ("Max CC"=w442:sgl, "CC Image Out"=w441:T4)  [unwired: 8 in, 1 out]
                n139 = Greater?(x=w442, y=w443) -> (0:w444:bool)
                n140 = case shown="True" w444 {
                  tunnel: w435 -> [_ w446]
                  tunnel: w441 -> [_ w445]
                  frame False {
                  }
                  frame True {
                    n141 = call "IMAQ Copy"("Image Dst"=w446, "Image Src"=w445) -> ()  [unwired: 4 in, 2 out]
                  }
                }
              }
              n142 = To Double Precision Float(number=w404) -> (double precision float=w403:dbl[])
              n143 = call "4Pi Focus Lock - Find Peak Position.vi"("Fit Size"=2, "y"=w403, "x"=w433) -> ("Peak value"=→"cc max":dbl, "Coerced Peak Position"=w428:dbl)  [unwired: 6 in, 1 out]
              "Measured Z (µm)" <- w428
              n144 = Not A Number/Path/Refnum?(number/path/refnum=w428) -> (NaN/Path/Refnum?=w427:bool)
              n145 = Select(t=4Pi_Focus_Lock_-_Actions."Get Current Position", s=w427, f=4Pi_Focus_Lock_-_Actions."Get Current XY Position" ("y")) -> (s? t:f=w424:T2)
            }
            frame "Get Current XY Position" {
              w463 = 3 ("edge size")
              n146 = Get Notifier Status(notifier=w453) -> (notifier out=w449:refnum<notifier>, current notification=w452:T3)  [unwired: 1 in, 3 out]
              n147 = Unbundle By Name(w452) -> ("CC Image Max (SGL)"=w473:T4)
              n148 = call "IMAQ ImageToArray"("Image"=w473) -> ("Image Pixels (Float)"=w460:sgl[][])  [unwired: 3 in, 4 out]
              n149 = call "4Pi Focus Lock - FFT shift 2D.vi"("Input image"=w460) -> ("fft shifted image"=w459:sgl[][])  [unwired: 10 in]
              n150 = call "4Pi Focus Lock - Crop Imag at Max.vi"("edge size"=w463, "Input array"=w459) -> ("Y"=w469:i32, "X"=w470:i32, "subarray"=w472:sgl[][])  [unwired: 6 in, 1 out]
              n151 = To Double Precision Float(number=w472) -> (double precision float=w455:dbl[][])
              n152 = Build Array(w470, w469) -> (w468:i32[])
              n153 = call "4Pi Focus Lock - 2D Gaussian - Fit -init.vi"("Image In (DBL)"=w455, "width"=10.0) -> ("Best Fit Params"=w471:T12)  [unwired: 12 in, 1 out]
              n154 = To Double Precision Float(number=w468) -> (double precision float=w465:dbl[])
              n155 = Unbundle By Name(w471) -> ("X Position"=w467:dbl, "Y Position"=w466:dbl)
              n156 = Build Array(w467, w466) -> (w464:dbl[])
              n157 = To Double Precision Float(number=w463) -> (double precision float=w462:dbl)
              n158 = Subtract(x=w464, y=w462) -> (x-y=w461:dbl[])
              n159 = Add(x=w461, y=w465) -> (x+y=w456:dbl[])
              n160 = Index Array(array=w456, index #1=0 ("index"), index #2=1 ("index")) -> (element #1=→"Measured X Position cc (px)":dbl, element #2=→"Measured Y Position cc (px)":dbl)
            }
            frame "Get Current Position 1" {
              n161 = Get Notifier Status(notifier=w493) -> (notifier out=w488:refnum<notifier>, current notification=w492:T3)  [unwired: 1 in, 3 out]
              n162 = Unbundle By Name(w492) -> ("No. of Frames"=w475:u32, "Cur Image (SGL)"=w477:T4, "CC Image (SGL)"=w483:T4)
              n163 = Unbundle By Name(w492) -> ("Sample Z (µm)"=w491:dbl[])
              n164 = Unbundle By Name(w492) -> ("Ref Stack (SGL)"=w486:T4[])
              n165 = To Unsigned Word Integer(number=w475) -> (unsigned 16bit integer=w474:u16)
              n166 = call "Generic Camera Get New Camera Image.vi"("Camera Notifier Name"=w478, "Frames"=w474) -> ("Image - U16"=w480:u16[][])  [unwired: 11 in, 2 out]
              n167 = To Single Precision Float(number=w480) -> (single precision float=w479:sgl[][])
              n168 = call "IMAQ ArrayToImage"("Image Pixels (Float)"=w479, "Image"=w477) -> ("Image Out"=w476:T4)  [unwired: 8 in, 1 out]
              n169 = call "4Pi Focus Lock - Img Norm.vi"("Image In"=w476) -> ("Image Dst Out"=w484:T4)  [unwired: 9 in, 1 out]
              n170 = for {
                tunnel: w486 -> [w504] mode=indexing
                tunnel: w484 -> [w502]
                tunnel: w483 -> [w501]
                tunnel: [w500] -> w482 mode=indexing
                n171 = call "4Pi Focus Lock - Img Norm.vi"("Image In"=w504) -> ("Image Dst Out"=w503:T4)  [unwired: 9 in, 1 out]
                n172 = call "IMAQ Multiply"("Image Src A"=w503, "Image Dst"=w501, "Image Src B"=w502) -> ("Image Dst Out"=w499:T4)  [unwired: 4 in, 1 out]
                n173 = call "IMAQ ImageToArray"("Image"=w499) -> ("Image Pixels (Float)"=w498:sgl[][])  [unwired: 3 in, 4 out]
                n174 = Add Array Elements(numeric array=w498) -> (sum=w496:sgl)
                n175 = Array Size(array=w498) -> (size(s)=w497:i32[])
                n176 = Multiply Array Elements(1:w497) -> (0:w495:i32)
                n177 = To Double Precision Float(number=w495) -> (double precision float=w494:dbl)
                n178 = Divide(x=w496, y=w494) -> (x/y=w500:dbl)
              }
              n179 = To Double Precision Float(number=w482) -> (double precision float=w485:dbl[])
              n180 = call "4Pi Focus Lock - Find Peak Position.vi"("Fit Size"=2, "y"=w485, "x"=w491) -> ("Coerced Peak Position"=w481:dbl)  [unwired: 6 in, 2 out]
              n181 = local write "Measured Z (µm)"(w481) -> ()
            }
            frame "Check Drift" {
              n182 = Get Notifier Status(notifier=w522) -> (notifier out=w515:refnum<notifier>, current notification=w521:T3)  [unwired: 1 in, 3 out]
              n183 = Unbundle By Name(w521) -> ("Z Correction Active"=w508:bool, "Z Drift Threshold"=w516:dbl, "PID Values"=w520:dbl[])
              n184 = local read "Measured Z (µm)"() -> (w511:dbl)
              n185 = local read "Target Z (µm)"() -> (w512:dbl)
              n186 = Array To Cluster(array=w520) -> (cluster=w519:T13)
              n187 = Subtract(x=w512, y=w511) -> (x-y=w513:dbl)
              n188 = call-poly <vilib>:"PID.vi"("PID gains"=w519, "process variable"=w511, "setpoint"=w512) -> ("dt out (s)"=→"dt (s)":dbl, "output"=→"dz (µm)":dbl)  [unwired: 7 in]
              n189 = Absolute Value(x=w513) -> (abs(x)=w510:dbl)
              n190 = Greater?(x=w510, y=w516) -> (0:w509:bool)
              n191 = And(x=w508, y=w509) -> (x .and. y?=w507:bool)
              n192 = case shown="True" w507 {
                tunnel: [4Pi_Focus_Lock_-_Actions."Update Plots" ("y") 4Pi_Focus_Lock_-_Actions."Move Z" ("y")] -> w505
                tunnel: [FALSE TRUE] -> w506
                frame False {
                }
                frame True {
                }
              }
              "Z Move" <- w506
            }
            frame "Move Z" {
              n193 = Get Notifier Status(notifier=w542) -> (notifier out=w535:refnum<notifier>, current notification=w541:T3)  [unwired: 1 in, 3 out]
              n194 = Unbundle By Name(w541) -> ("Z Stage Move Limit (µm)"=w539:dbl)
              n195 = local read "dz (µm)"() -> (w540:dbl)
              n196 = Multiply(x=w540, y="Update Scale Factor") -> (x*y=w533:dbl)
              n197 = Absolute Value(x=w533) -> (abs(x)=w538:dbl)
              n198 = Greater?(x=w539, y=w538) -> (0:w529:bool)
              n199 = local read "Z Move"() -> (w531:bool)
              n200 = And(x=w529, y=w531) -> (x .and. y?=w532:bool)
              n201 = case shown="True" w532 {
                tunnel: w533 -> [_ w544]
                tunnel: w537 -> [_ w543]
                frame False {
                }
                frame True {
                  n202 = Build Array(w544) -> (w545:dbl[])
                  n203 = flat-sequence {
                    tunnel: w545 -> [w551]
                    tunnel: w543 -> [w547]
                    frame #0 {
                      n204 = call "Stages Messenger.vi"("Stage Notifier Name"=w547, "Actions"=Stage_Actions."MVR", "Setpoint"=w551, "Axis"=bool[] [TRUE], "Exit While Busy?"=FALSE) -> ("Positions"=w549:dbl[])  [unwired: 7 in, 3 out]
                      n205 = Index Array(array=w549, index=0) -> ()  [unwired: 1 out]
                    }
                    frame #1 {
                      n206 = Wait (ms)(milliseconds to wait=u32 350) -> ()  [unwired: 1 out]
                    }
                  }
                }
              }
              n207 = Select(t=4Pi_Focus_Lock_-_Actions."Update Plots" ("y"), s=w529, f=4Pi_Focus_Lock_-_Actions."Abort") -> (s? t:f=w527:T2)
            }
            frame "Update Plots" {
              n208 = Get Notifier Status(notifier=w585) -> (notifier out=w573:refnum<notifier>, current notification=w583:T3)  [unwired: 1 in, 3 out]
              n209 = Unbundle By Name(w583) -> ("Z Drift Threshold"=w584:dbl)
              n210 = Unbundle By Name(w583) -> ("Initial Z Position (µm)"=w582:dbl)
              n211 = call "Stages Messenger.vi"("Stage Notifier Name"=w575, "Actions"=Stage_Actions."Get Position", "Exit While Busy?"=TRUE) -> ("Positions"=w576:dbl[])  [unwired: 9 in, 3 out]
              n212 = local read "Measured Z (µm)"() -> (w586:dbl)
              n213 = local read "Target Z (µm)"() -> (w587:dbl)
              n214 = Index Array(array=w576, index=0) -> (element=w574:dbl)
              n215 = local write "Stage Position (µm)"(w574) -> ()
              n216 = Subtract(x=w574, y=w582) -> (x-y=w581:dbl)
              n217 = call "4Pi Focus Lock - Values Organize Plot Data.vi"("Target 01"=w587, "Value Limit"=w584, "Current 01"=w586, "Stage Position"=w581) -> ("output cluster"=→"Z Target and Fit Value (µm)":T1)  [unwired: 11 in]
              n218 = local read "Measured X Position cc (px)"() -> (w565:dbl)
              n219 = local read "Measured Y Position cc (px)"() -> (w564:dbl)
              n220 = local read "Target X Position cc (px)"() -> (w563:dbl)
              n221 = local read "Target Y Position cc (px)"() -> (w562:dbl)
              n222 = Build Array(w565, w564) -> (w569:dbl[])
              n223 = Build Array(w563, w562) -> (w570:dbl[])
              n224 = Subtract(x=w569, y=w570) -> (x-y=w561:dbl[])
              n225 = Multiply(x=w561, y="Pixe Size (µm)") -> (x*y=w568:dbl[])
              n226 = local read "cc max"() -> (w555:dbl)
              n227 = Index Array(array=w568, index #1=0 ("index"), index #2=1 ("index")) -> (element #1=w560:dbl, element #2=w559:dbl)
              n228 = Bundle(w560, w559, 0.0) -> (→"X Y Fit Value (µm)":cluster{dbl, dbl, dbl})  [unwired: 1 in]
              n229 = Bundle("cc max"=w555) -> (→"CC Max":cluster{" cc max":dbl})  [unwired: 1 in]
            }
            frame "Abort" {
              n230 = Get Notifier Status(notifier=w593) -> (notifier out=w598:refnum<notifier>, current notification=w597:T3)  [unwired: 1 in, 3 out]
              n231 = call "Camera Messenger.vi"("Notifier Name"=w592, "General Camera Actions"=Generic_Camera_Actions."Abort") -> ()  [unwired: 8 in, 6 out]
              n232 = Bundle By Name(cluster=w597, "Running?"=FALSE, "Actions"=4Pi_Focus_Lock_-_Actions."Exit Loop") -> (w595:T3)
              n233 = Send Notification(notification=w595, notifier=w598) -> (notifier out=w589:refnum<notifier>)  [unwired: 1 in, 1 out]
            }
            frame "Exit Loop" {
            }
            frame "Quit" {
              n234 = Get Notifier Status(notifier=w603) -> (current notification=w609:T3)  [unwired: 1 in, 4 out]
              n235 = Unbundle By Name(w609) -> ("Ref Stack (SGL)"=w608:T4[], "Cur Image (SGL)"=w607:T4, "Tmp Image FFT (CSG)"=w606:T4[], "CC Image (SGL)"=w605:T4, "Ref FFT Stack (CSG)"=w602:T4[])
              n236 = Build Array (concatenate)(w608, w607, w606, w605, w602) -> (w604:T4[])
              n237 = for {
                tunnel: w604 -> [w612] mode=indexing
                n238 = call "IMAQ Dispose"("Image"=w612) -> ()  [unwired: 5 in, 1 out]
              }
            }
          }
          n239 = Get Notifier Status(notifier=w217) -> (current notification=w225:T3)  [unwired: 1 in, 4 out]
          n240 = Unbundle By Name(w225) -> ("Actions"=w224:T2)
          n241 = Equal?(x=w222, y=w224) -> (x = y?=w223:bool)
          n242 = Select(t=w222, s=w223, f=w221) -> (s? t:f=w220:T2)
        }
      }
      n243 = while {
        tunnel: w73 -> [w89]
        tunnel: w72 -> [w88]
        stop <- w87 stop-if-true
        n244 = event shown="[4] \"Z Correction Active\": Value Change" {
          selector: _ -> [_ _ _ _ _ _ _]
          dyn-events: _ -> [_ _ _ _ _ _ _]
          timeout: -1 -> [_ _ _ _ _ _ _]
          tunnel: w89 -> [_ w92 _ _ _ _ _]
          tunnel: w88 -> [_ _ w102 w140 w167 w178 w182]
          tunnel: [w90 w91 w93 w137 _ w172 w180] -> w87
          tunnel: FALSE ("NewVal") -> [w90 w91 w93 w137 _ w172 _]
          event Timeout {
            n245 = event-data() -> ()  [unwired: 1 in, 3 out]
          }
          event "Set Camera ROI": Value Change {
            n246 = event-data() -> ()  [unwired: 1 in, 2 out]
            n247 = call "4Pi Focus Lock - Setup Camera.vi"("Camera Notifier Name"=w92) -> ()  [unwired: 14 in, 1 out]
          }
          event "P (Proportional)", "I (Integral)", "D (Derivative)", "Sample Z Step Size (µm)", "Z Move Limit (µm)", "Z Drift Threshold (µm)": Value Change {
            n248 = event-data() -> ("NewVal"=w97:dbl, "CtlRef"=w99:refnum<vi>)  [unwired: 1 in]
            n249 = Get Notifier Status(notifier=w102) -> (notifier out=w101:refnum<notifier>, current notification=w100:T3)  [unwired: 1 in, 3 out]
            n250 = property class="DigNum (strict)"(reference=w99) -> ("Label.Text"=w98:string)  [unwired: 1 in, 2 out]
            n251 = case shown="Default" w98 {
              tunnel: w100 -> [w103 w106 w112 w118 w124 w127 w130]
              tunnel: w97 -> [_ w107 w113 w119 w123 w126 w129]
              tunnel: [w103 w104 w110 w116 w122 w125 w128] -> w96
              frame Default {
              }
              frame "P (Proportional)" {
                n252 = Unbundle By Name(w106) -> ("PID Values"=w108:dbl[])
                n253 = Replace Array Subset(array=w108, new element=w107, index=0) -> (w105:dbl[])
                n254 = Bundle By Name(cluster=w106, "PID Values"=w105) -> (w104:T3)
              }
              frame "I (Integral)" {
                n255 = Unbundle By Name(w112) -> ("PID Values"=w114:dbl[])
                n256 = Replace Array Subset(array=w114, new element=w113, index=1) -> (w111:dbl[])
                n257 = Bundle By Name(cluster=w112, "PID Values"=w111) -> (w110:T3)
              }
              frame "D (Derivative)" {
                n258 = Unbundle By Name(w118) -> ("PID Values"=w120:dbl[])
                n259 = Replace Array Subset(array=w120, new element=w119, index=2) -> (w117:dbl[])
                n260 = Bundle By Name(cluster=w118, "PID Values"=w117) -> (w116:T3)
              }
              frame "Sample Z Step Size (µm)" {
                n261 = Bundle By Name(cluster=w124, "Z Step Size (µm)"=w123) -> (w122:T3)
              }
              frame "Z Move Limit (µm)" {
                n262 = Bundle By Name(cluster=w127, "Z Stage Move Limit (µm)"=w126) -> (w125:T3)
              }
              frame "Z Drift Threshold (µm)" {
                n263 = Bundle By Name(cluster=w130, "Z Drift Threshold"=w129) -> (w128:T3)
              }
            }
            n264 = Bundle By Name(cluster=w96, "Actions"=4Pi_Focus_Lock_-_Actions."Idle") -> (w94:T3)
            n265 = Send Notification(notification=w94, notifier=w101) -> ()  [unwired: 1 in, 2 out]
          }
          event "Sample Z Step No.", "Frame Accumulation": Value Change {
            n266 = event-data() -> ("NewVal"=w136:u32, "CtlRef"=w132:refnum<vi>)  [unwired: 1 in]
            n267 = property class="DigNum (strict)"(reference=w132) -> ("Label.Text"=w131:string)  [unwired: 1 in, 2 out]
            n268 = Get Notifier Status(notifier=w140) -> (notifier out=w138:refnum<notifier>, current notification=w139:T3)  [unwired: 1 in, 3 out]
            n269 = case shown="\"Frame Accumulation\"" w131 {
              tunnel: w139 -> [w141 w146 w161]
              tunnel: [w141 w145 w159] -> w135
              tunnel: w136 -> [_ w144 w160]
              frame Default {
              }
              frame "Sample Z Step No." {
                n270 = for {
                  N: w144 -> [_]
                  tunnel: [w158] -> w143 mode=indexing
                  tunnel: [w147] -> w142 mode=indexing
                  i -> [w157]
                  w148 = T5 3 items=["Grayscale (U8)", "Grayscale (I16)", "Grayscale (SGL)", "Complex (CSG)", "RGB (U32)", "HSL (U32)", "RGB (U64)", "Grayscale (U16)"] ("Image Type")
                  w153 = T5 2 items=["Grayscale (U8)", "Grayscale (I16)", "Grayscale (SGL)", "Complex (CSG)", "RGB (U32)", "HSL (U32)", "RGB (U64)", "Grayscale (U16)"] ("Image Type")
                  w149 = 10 ("Border Size")
                  n271 = Number To Decimal String(number=w157, width (-)=i16 1) -> (decimal integer string=w155:string)
                  n272 = Concatenate Strings("Ref Stack " ("string"), w155) -> (w151:string)
                  n273 = call "IMAQ Create"("Border Size"=w149, "Image Name"=w151, "Image Type"=w153) -> ("New Image"=w158:T4)  [unwired: 2 in, 1 out]
                  n274 = Concatenate Strings("FFT" ("string"), w151) -> (w150:string)
                  n275 = call "IMAQ Create"("Border Size"=w149, "Image Name"=w150, "Image Type"=w148) -> ("New Image"=w147:T4)  [unwired: 2 in, 1 out]
                }
                n276 = Bundle By Name(cluster=w146, "Z Step No."=w144, "Ref Stack (SGL)"=w143, "Ref FFT Stack (CSG)"=w142) -> (w145:T3)
              }
              frame "Frame Accumulation" {
                n277 = Bundle By Name(cluster=w161, "No. of Frames"=w160) -> (w159:T3)
              }
            }
            n278 = Bundle By Name(cluster=w135, "Actions"=4Pi_Focus_Lock_-_Actions."Idle") -> (w133:T3)
            n279 = Send Notification(notification=w133, notifier=w138) -> ()  [unwired: 1 in, 2 out]
          }
          event "Z Correction Active": Value Change {
            n280 = event-data() -> ("NewVal"=w165:bool)  [unwired: 1 in, 1 out]
            n281 = Get Notifier Status(notifier=w167) -> (notifier out=w163:refnum<notifier>, current notification=w166:T3)  [unwired: 1 in, 3 out]
            n282 = Bundle By Name(cluster=w166, "Actions"=4Pi_Focus_Lock_-_Actions."Idle", "Z Correction Active"=w165) -> (w162:T3)
            n283 = Send Notification(notification=w162, notifier=w163) -> ()  [unwired: 1 in, 2 out]
          }
          event "Start Lock": Value Change {
            n284 = event-data() -> ("NewVal"=w170:bool)  [unwired: 1 in]
            n285 = Select(t=4Pi_Focus_Lock_-_Actions."Start Lock", s=w170, f=4Pi_Focus_Lock_-_Actions."Abort" ("t")) -> (s? t:f=w175:T2)
            n286 = Select(t=TRUE ("Running?"), s=w170, f=FALSE) -> (s? t:f=w168:bool)
            n287 = Get Notifier Status(notifier=w178) -> (notifier out=w179:refnum<notifier>, current notification=w177:T3)  [unwired: 1 in, 3 out]
            n288 = Bundle By Name(cluster=w177, "Actions"=w175, "Running?"=w168) -> (w176:T3)
            n289 = Send Notification(notification=w176, notifier=w179) -> ()  [unwired: 1 in, 2 out]
          }
          event "Quit": Value Change {
            # "Turn off the Focus lock before quiting."
            n290 = event-data() -> ("NewVal"=w180:bool)  [unwired: 1 in]
            n291 = Get Notifier Status(notifier=w182) -> (notifier out=w185:refnum<notifier>, current notification=w183:T3)  [unwired: 1 in, 3 out]
            n292 = Unbundle By Name(w183) -> ("Running?"=w186:bool)
            n293 = case shown="False" w186 {
              tunnel: w185 -> [w190 w195]
              tunnel: [w190 w192] -> w184
              tunnel: w183 -> [_ w196]
              frame False {
              }
              frame True {
                n294 = Bundle By Name(cluster=w196, "Actions"=4Pi_Focus_Lock_-_Actions."Abort") -> (w194:T3)
                n295 = Send Notification(notification=w194, notifier=w195) -> (notifier out=w193:refnum<notifier>)  [unwired: 1 in, 1 out]
                n296 = while {
                  tunnel: w193 -> [w206]
                  tunnel: [w201] -> w192
                  i -> [w200]
                  stop <- w202 stop-if-true
                  n297 = Get Notifier Status(notifier=w206) -> (notifier out=w201:refnum<notifier>, # waiting=w205:i32)  [unwired: 1 in, 3 out]
                  n298 = Greater?(x=w200, y=1500) -> (0:w198:bool)
                  n299 = Less?(x=w205, y=1) -> (x < y?=w203:bool)
                  n300 = Or(x=w203, y=w198) -> (x .or. y?=w202:bool)
                  n301 = Wait (ms)(milliseconds to wait=u32 1) -> ()  [unwired: 1 out]
                }
              }
            }
            n302 = Get Notifier Status(notifier=w184) -> (notifier out=w188:refnum<notifier>, current notification=w189:T3)  [unwired: 1 in, 3 out]
            n303 = Bundle By Name(cluster=w189, "Actions"=4Pi_Focus_Lock_-_Actions."Quit") -> (w187:T3)
            n304 = Send Notification(notification=w187, notifier=w188) -> ()  [unwired: 1 in, 2 out]
          }
        }
      }
      n305 = Release Notifier(notifier=w70, force destroy? (F)=TRUE) -> ()  [unwired: 1 in, 3 out]
    }
    frame Error {
    }
  }
